vi "Update Flow.vi"(8 "error in":errorcluster, 9 "Status":map{string, bool}(c390), 10 "Flow":sgl, 11 "DeepU Results in":refnum<class "DeepU Results.lvclass">) -> (0 "error out":errorcluster, 3 "DeepU Results out":refnum<class "DeepU Results.lvclass">)   [LabVIEW 2019, in "Results.lvlib" / "DeepU Results.lvclass"]
uses:
  DeepU Results.lvclass
  DeepU Results.lvclass/DeepU Results.ctl
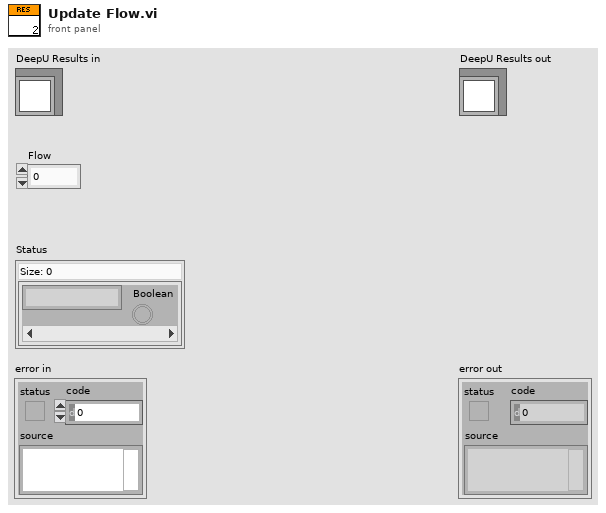
[diagram p1: front panel]
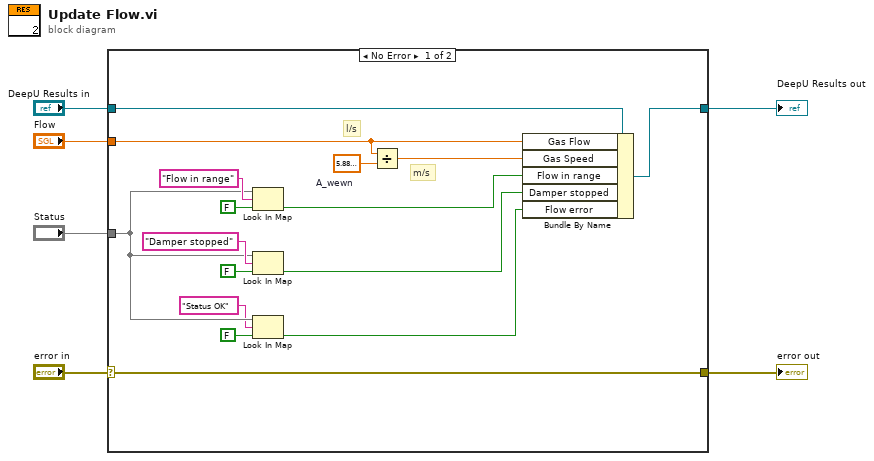
[diagram p0: block diagram]
diagram:
  n1 = case shown="No Error" "error in" {
    selector: "error in" -> [w21 w24]
    tunnel: [w21 w24] -> w5
    tunnel: [w20 w23] -> w3
    tunnel: "DeepU Results in" -> [w22 w23]
    tunnel: "Flow" -> [w8 _]
    tunnel: "Status" -> [w15 _]
    frame No Error {
      w7 = sgl 5.89  # A_wewn
      # "m/s"
      # "l/s"
      n2 = Look In Map(map=w15, key="Flow in range", default value=FALSE) -> (value=w18:bool)  [unwired: 1 out]
      n3 = Look In Map(map=w15, key="Damper stopped", default value=FALSE) -> (value=w16:bool)  [unwired: 1 out]
      n4 = Look In Map(map=w15, key="Status OK", default value=FALSE) -> (value=w13:bool)  [unwired: 1 out]
      n5 = Divide(x=w8, y=w7) -> (x/y=w9:sgl)
      n6 = Bundle By Name(cluster=w22, "Gas Flow"=w8, "Gas Speed"=w9, "Flow in range"=w18, "Damper stopped"=w16, "Flow error"=w13) -> (w20:refnum<class "DeepU Results.lvclass">)
    }
    frame Error {
    }
  }
  "error out" <- w5
  "DeepU Results out" <- w3
